vi "RedistributeArmPathPoints.vi"(1 "Desired Point Spacing (in)":dbl, 2 "Path Length (in)":dbl, 3 "ArmPathIn":T1[](array[typedef]), 4 "IndexedPathLength":dbl[](array[numeric])) -> (0 "ArmPathOut":T1[](array[typedef]))   [LabVIEW 2017]
uses:
  TypeDefs/ArmCoordinate.ctl
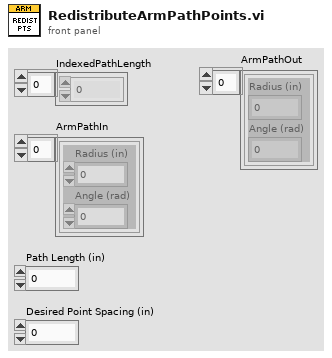
[diagram p1: front panel]
types:
  T1 = typedef "ArmCoordinate.ctl" = cluster{"Radius (in)":dbl, "Angle (rad)":dbl}
  T2 = typedef "Point2D.ctl" = cluster{"X":dbl, "Y":dbl}
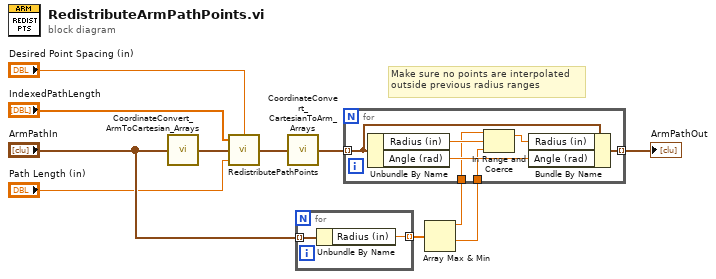
[diagram p0: block diagram]
diagram:
  # "Make sure no points are interpolated\noutside previous radius ranges"
  n1 = call "CoordinateConvert_ArmToCartesian_Arrays.vi"("ArmCoordinates"="ArmPathIn") -> ("XYPoints"=w4:T2[])
  n2 = call "RedistributePathPoints.vi"("Desired Point Spacing (in)"="Desired Point Spacing (in)", "Path Length (in)"="Path Length (in)", "PathIn"=w4, "IndexedPathLength"="IndexedPathLength") -> ("PathOut"=w5:T2[])
  n3 = call "CoordinateConvert_CartesianToArm_Arrays.vi"("XYPoints"=w5) -> ("ArmCoordinates"=w9:T1[])
  n4 = for {
    tunnel: "ArmPathIn" -> [w13] mode=indexing
    tunnel: [w12] -> w11 mode=indexing
    n5 = Unbundle By Name(w13) -> ("Radius (in)"=w12:dbl)
  }
  n6 = Array Max & Min(array=w11) -> (max value=w7:dbl, min value=w6:dbl)  [unwired: 2 out]
  n7 = for {
    tunnel: w9 -> [w19] mode=indexing
    tunnel: [w20] -> w8 mode=indexing
    tunnel: w7 -> [w15]
    tunnel: w6 -> [w14]
    n8 = Unbundle By Name(w19) -> ("Radius (in)"=w16:dbl, "Angle (rad)"=w18:dbl)
    n9 = In Range and Coerce(upper limit=w15, x=w16, lower limit=w14) -> (coerced(x)=w17:dbl)  [unwired: 1 out]
    n10 = Bundle By Name(cluster=w19, "Radius (in)"=w17, "Angle (rad)"=w18) -> (w20:T1)
  }
  "ArmPathOut" <- w8
